vi "RemoteVI Frame Encode.vi"(0 "seq":u32, 5 "width":u16, 7 "height":u16, 9 "rects":cluster{"x":i16, "y":i16, "png":string}[](array[cluster])) -> (4 "message":string)   [LabVIEW 2020, in "RemoteVI.lvlib"]
doc: "Encodes one RemoteVI protocol v2 FRAME message (docs/protocol.md). Layout, all integers big-endian: 0x52, 0x01, seq U32, width U16, height U16, rect count U16, then per rect x I16, y I16, png length U32 and the png bytes. Pure function, cannot fail. Reference: encodeFrame() in tools\\lib\\protocol.mjs."
uses:
  RemoteVI.lvlib
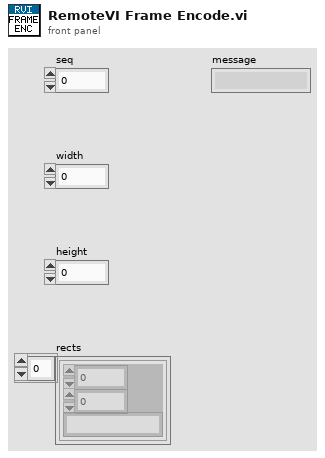
[diagram p1: front panel]
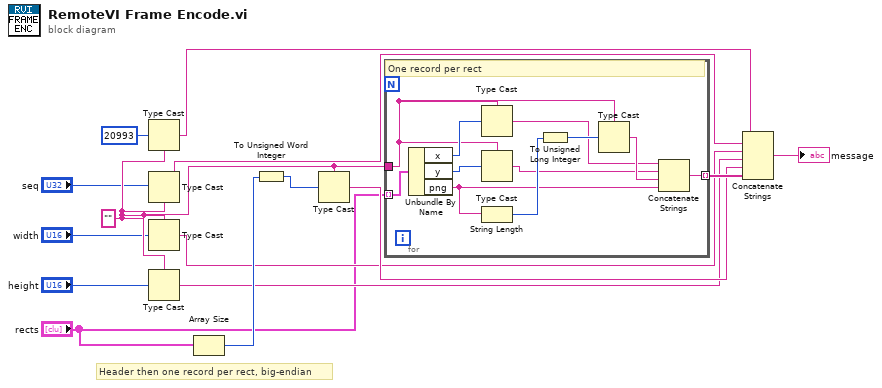
[diagram p0: block diagram]
diagram:
  w6 = ""
  # "Header then one record per rect, big-endian"
  n1 = Type Cast(type=w6, x=u16 20993) -> (*(type *) &x=w7:string)
  n2 = Type Cast(type=w6, x="seq") -> (*(type *) &x=w8:string)
  n3 = Type Cast(type=w6, x="width") -> (*(type *) &x=w9:string)
  n4 = Type Cast(type=w6, x="height") -> (*(type *) &x=w10:string)
  n5 = Array Size(array="rects") -> (size(s)=w11:i32)
  n6 = To Unsigned Word Integer(number=w11) -> (unsigned 16bit integer=w12:u16)
  n7 = Type Cast(type=w6, x=w12) -> (*(type *) &x=w13:string)
  n8 = for {
    tunnel: "rects" -> [w16] mode=indexing
    tunnel: w6 -> [w17]
    tunnel: [w26] -> w14 mode=indexing
    # "One record per rect"
    n9 = Unbundle By Name(w16) -> ("x"=w18:i16, "y"=w19:i16, "png"=w20:string)
    n10 = Type Cast(type=w17, x=w18) -> (*(type *) &x=w21:string)
    n11 = Type Cast(type=w17, x=w19) -> (*(type *) &x=w22:string)
    n12 = String Length(string=w20) -> (length=w23:i32)
    n13 = To Unsigned Long Integer(number=w23) -> (unsigned 32bit integer=w24:u32)
    n14 = Type Cast(type=w17, x=w24) -> (*(type *) &x=w25:string)
    n15 = Concatenate Strings(w21, w22, w25, w20) -> (w26:string)
  }
  n16 = Concatenate Strings(w7, w8, w9, w10, w13, w14) -> (→"message":string)
